vi "Clear References.vi"(8 "error in (no error)":errorcluster, 11 "Dialog in":refnum<class "Dialog.lvclass">) -> (0 "error out":errorcluster, 3 "Dialog out":refnum<class "Dialog.lvclass">)   [LabVIEW 2012, in "Dialog.lvlib" / "Dialog.lvclass"]
uses:
  Dialog.lvclass
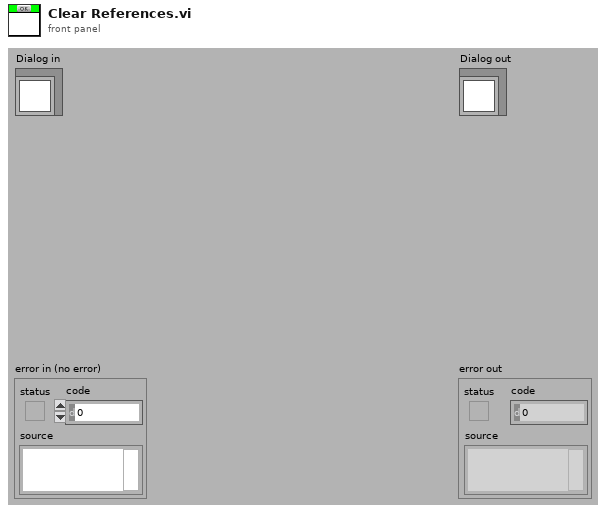
[diagram p1: front panel]
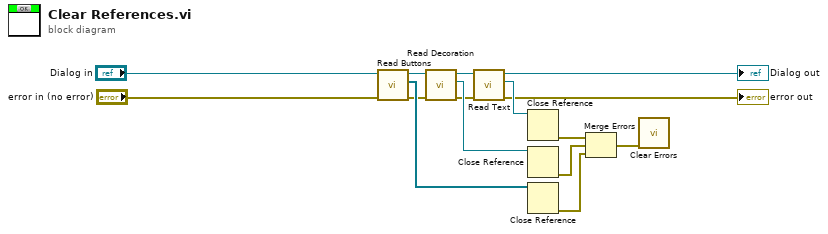
[diagram p0: block diagram]
diagram:
  n1 = call-dynamic "Read Buttons.vi"("error in (no error)"="error in (no error)", "Dialog.lvclass in"="Dialog in") -> ("error out"=w4:errorcluster, "Buttons"=w11:refnum<vi>[], "Dialog.lvclass out"=w13:refnum<class "Dialog.lvclass">)  [unwired: 7 out]
  n2 = call-dynamic "Read Decoration.vi"("error in (no error)"=w4, "Dialog.lvclass in"=w13) -> ("error out"=w3:errorcluster, "Decoration"=w10:refnum<vi>, "Dialog.lvclass out"=w12:refnum<class "Dialog.lvclass">)  [unwired: 7 out]
  n3 = call-dynamic "Read Text.vi"("error in (no error)"=w3, "Dialog.lvclass in"=w12) -> ("error out"=→"error out":errorcluster, "Text"=w9:refnum<vi>, "Dialog.lvclass out"=→"Dialog out":refnum<class "Dialog.lvclass">)  [unwired: 7 out]
  n4 = Close Reference(reference=w9) -> (error out=w7:errorcluster)  [unwired: 1 in]
  n5 = Close Reference(reference=w10) -> (error out=w6:errorcluster)  [unwired: 1 in]
  n6 = Close Reference(reference=w11) -> (error out=w5:errorcluster)  [unwired: 1 in]
  n7 = Merge Errors(w7, w6, w5) -> (w8:errorcluster)
  n8 = call <vilib>:"Clear Errors.vi"("error in (no error)"=w8) -> ()  [unwired: 7 out]
